vi "Close VI Reference.vi"(8 "error in":errorcluster, 11 "ILabVIEWFile in":refnum<class "Type Definition.lvclass">) -> (0 "error out":errorcluster, 3 "ILabVIEWFile out":refnum<class "Type Definition.lvclass">)   [LabVIEW 2026, in "Type Definition.lvclass"]
doc: "Close all VI/element references of the object."
uses:
  Type Definition.lvclass
  Type Definition.lvclass/Type Definition.ctl
  LabVIEW File/LabVIEW File.lvclass
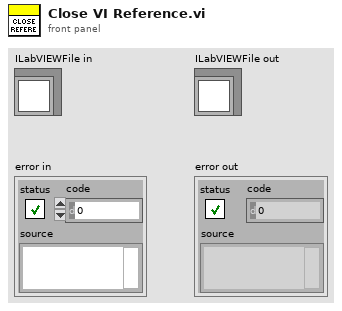
[diagram p1: front panel]
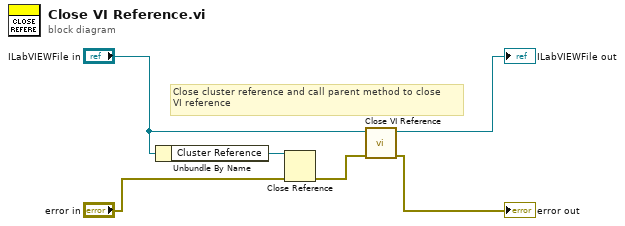
[diagram p0: block diagram]
diagram:
  # "Close cluster reference and call parent method to close\nVI reference"
  n1 = Unbundle By Name("ILabVIEWFile in") -> ("Cluster Reference"=w3:refnum<vi>)
  n2 = Close Reference(reference=w3, error in (no error)="error in") -> (error out=w5:errorcluster)
  n3 = call-parent "Close VI Reference.vi"("error in"=w5, "ILabVIEWFile in"="ILabVIEWFile in") -> ("error out"=→"error out":errorcluster, "ILabVIEWFile out"=→"ILabVIEWFile out":refnum<class "Type Definition.lvclass">)  [unwired: 8 in]
